vi "Create Client.vi"(8 "error in":errorcluster, 10 "Server Certificate File (.crt)":path, 11 "address":string) -> (0 "error out":errorcluster, 3 "gRPC ID Out":T1)   [LabVIEW 2021, in "CAN_Reader_CANsub_Wrapper.lvlib"]
uses:
  CAN_Reader_CANsub_Wrapper.lvlib
  <vilib>/gRPC/LabVIEW gRPC Library/grpc-lvsupport-release.lvlib
  <vilib>/CIF Foundation/CIF Core/CIFUtilities/CIFConfigurationFile/CIF Configuration File.lvlib
  <vilib>/CIF Foundation/CIF Core/CIFCore/Grpc/CIFCorePlugin_client/CIFCorePlugin_client.lvlib
  <vilib>/CIF Foundation/CIF Core/CIFCore/Grpc/CIFCoreChannel_client/CIFCoreChannel_client.lvlib
  CanReaderCansub_client/CanReaderCansub_client.lvlib
  <vilib>/CIF Foundation/CIF U8 Array Monitor gRPC/U8_Array_Monitor_gRPC/CIFU8ArrayMonitor_client/CIFU8ArrayMonitor_client.lvlib
  <vilib>/gRPC/LabVIEW gRPC Library/Shared/grpcId.ctl
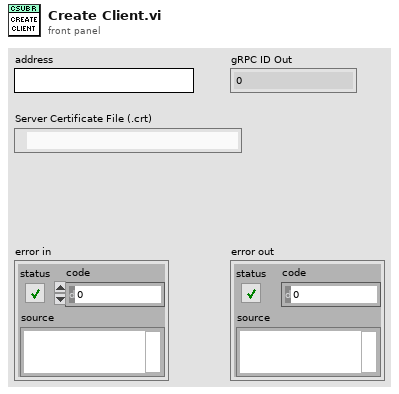
[diagram p1: front panel]
types:
  T1 = typedef "grpc-lvsupport-release.lvlib/grpcId.ctl" = u64
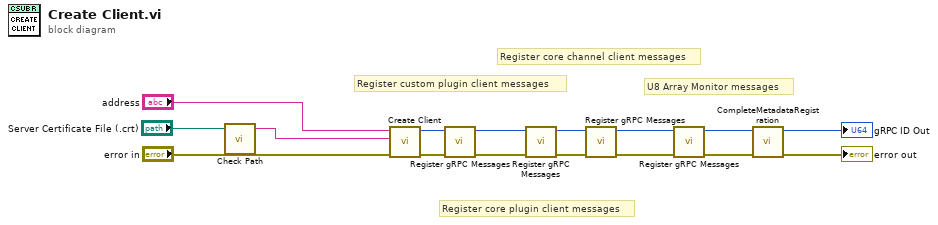
[diagram p0: block diagram]
diagram:
  # "U8 Array Monitor messages"
  # "Register core channel client messages"
  # "Register core plugin client messages"
  # "Register custom plugin client messages"
  n1 = call <vilib>:"Check Path.vi"("path"="Server Certificate File (.crt)") -> ("Path String"=w9:string)  [unwired: 3 in]
  n2 = call <vilib>:"Create Client.vi"("error in"="error in", "certificate path"=w9, "address"="address") -> ("error out"=w11:errorcluster, "ClientID out"=w12:T1)  [unwired: 7 in]
  n3 = call <vilib>:"Register gRPC Messages.vi"("error in (no error)"=w11, "gRPC ID"=w12) -> ("error out"=w5:errorcluster, "gRPC ID Out"=w6:T1)  [unwired: 8 in]
  n4 = call <vilib>:"Register gRPC Messages.vi"("error in (no error)"=w5, "gRPC ID"=w6) -> ("error out"=w8:errorcluster, "gRPC ID Out"=w7:T1)  [unwired: 8 in]
  n5 = call <vilib>:"Register gRPC Messages.vi"("error in (no error)"=w8, "gRPC ID"=w7) -> ("error out"=w3:errorcluster, "gRPC ID Out"=w4:T1)  [unwired: 8 in]
  n6 = call <vilib>:"Register gRPC Messages.vi"("error in (no error)"=w3, "gRPC ID"=w4) -> ("error out"=w2:errorcluster, "gRPC ID Out"=w1:T1)  [unwired: 8 in]
  n7 = call <vilib>:"CompleteMetadataRegistration.vi"("error in"=w2, "gRPC ID in"=w1) -> ("error out"=→"error out":errorcluster, "gRPC ID Out"=→"gRPC ID Out":T1)  [unwired: 8 in]
